vi "Start.vi"(8 "error in (no error)":errorcluster, 10 "Container":refnum<vi>, 11 "ArrayManager in":refnum<class "ArrayManager.lvclass">) -> (0 "error out":errorcluster, 3 "ArrayManager out":refnum<class "ArrayManager.lvclass">)   [LabVIEW 2020, in "OOPanel.lvlib" / "ArrayManager.lvclass"]
uses:
  ArrayManager.lvclass
  ArrayManager.lvclass/ArrayManager.ctl
  Array Panel Async.vi
  lv-exec-anchor/ExecAnchor/ExecAnchor.lvclass
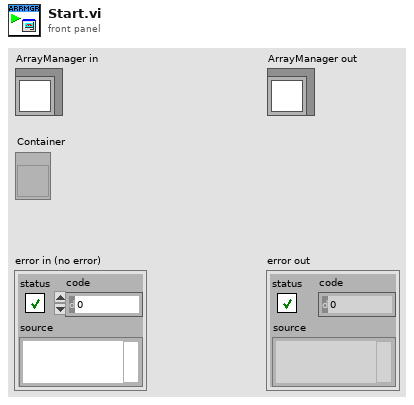
[diagram p1: front panel]
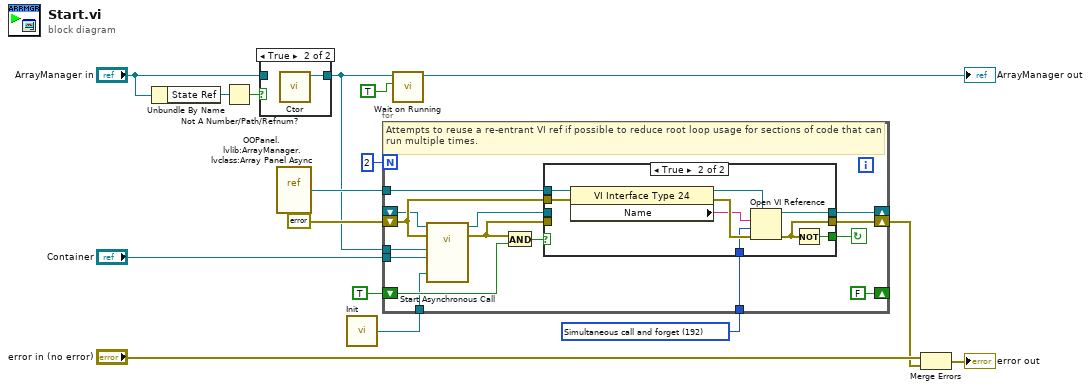
[diagram p0: block diagram]
diagram:
  w7 = 192 items=["Record modifications"=1, "Open templates for editing"=2, "Prompt user to save"=4, "Prepare for reentrant run"=8, "Prompt to find missing subVIs"=16, "Hide loading dialog box"=32, "Enable simultaneous calls"=64, "Prepare to call and forget"=128, "Simultaneous call and forget"=192, "Prepare to call and collect"=256, "Simultaneous call and collect"=320]
  n1 = Unbundle By Name("ArrayManager in") -> ("State Ref"=w12:refnum<data-value>)
  n2 = Not A Number/Path/Refnum?(number/path/refnum=w12) -> (NaN/Path/Refnum?=w11:bool)
  n3 = case shown="True" w11 {
    tunnel: "ArrayManager in" -> [w17 _]
    tunnel: [w17 w18] -> w5
    frame False {
    }
    frame True {
      n4 = call "Ctor.vi"() -> ("PanelArray"=w18:refnum<class "ArrayManager.lvclass">)  [unwired: 10 in, 1 out]
    }
  }
  n5 = vi-ref "OOPanel.lvlib:ArrayManager.lvclass:Array Panel Async.vi"() -> (w6:refnum<vi>)
  n6 = call "Init.vi"() -> ("ExecAnchor out"=w1:refnum<class "ExecAnchor.lvclass">)  [unwired: 7 in]
  n7 = for {
    N: 2 -> [_]
    tunnel: w6 -> [w32]
    tunnel: w7 -> [w31]
    shift-right: [w30] -> _
    shift-left: _ -> [w29]
    shift-right: [w27] -> w3
    shift-left: errorcluster {"status"=FALSE, "code"=0, "source"=""} ("error constant") -> [w33]
    shift-right: [FALSE] -> _
    shift-left: TRUE -> [w24]
    tunnel: w5 -> [w21]
    tunnel: "Container" -> [w20]
    tunnel: w1 -> [w19]
    stop <- w23 continue-if-true
    # "Attempts to reuse a re-entrant VI ref if possible to reduce root loop usage for sections of code that can run multiple times."
    n8 = call-by-ref "Start Asynchronous Call"(reference=w29, error in=w33, "ExecAnchor"=w19, "Container"=w20, "PanelArray in"=w21) -> (reference out=w28:refnum<vi>, error out=w26:errorcluster)  [unwired: 9 in]
    n9 = And(x=w26, y=w24) -> (x .and. y?=w25:bool)
    n10 = case shown="True" w25 {
      tunnel: w32 -> [_ w43]
      tunnel: w31 -> [_ w41]
      tunnel: [w35 w39] -> w30
      tunnel: w28 -> [w35 _]
      tunnel: [w34 w37] -> w27
      tunnel: w26 -> [w34 _]
      tunnel: w33 -> [_ w38]
      tunnel: [_ w36] -> w23
      frame False {
      }
      frame True {
        n11 = property class="VI Interface Type 24"(reference=w43, error in=w38) -> (reference out=w40:refnum<vi>, error out=w44:errorcluster, "Name"=w42:string)
        n12 = Open VI Reference(type specifier VI Refnum (for type only)=w40, vi path=w42, options=w41, error in (no error)=w44) -> (vi reference=w39:refnum<vi>, error out=w37:errorcluster)  [unwired: 2 in]
        n13 = Not(x=w37) -> (.not. x?=w36:bool)
      }
    }
  }
  n14 = call "Wait on Running.vi"("Value"=TRUE, "ArrayManager in"=w5) -> ("ArrayManager out"=→"ArrayManager out":refnum<class "ArrayManager.lvclass">)  [unwired: 8 in, 1 out]
  n15 = Merge Errors("error in (no error)", w3) -> (→"error out":errorcluster)
